vi "Transfer Images Data to UI.vi"(0 "fpga interface in":refnum<k20>, 1 "'stop' notifier":refnum<notifier>, 2 "Auto Vision Config":T1, 3 "measure call context in":refnum<class "Measure Call Context.lvclass">, 5 "Active Channel":string[](array[string]), 11 "error in":errorcluster, 12 "References":T6, 13 "raw display notifier":refnum<notifier>) -> (4 "fpga interface out":refnum<k20>, 15 "error out":errorcluster)   [LabVIEW 2025, in "Automotive Vision.lvclass"]
doc: "Handles frame grabbing, and prepare data for sendig it to the UI."
uses:
  Automotive Vision.lvclass
  <vilib>/Plug-In SDKs/Measurements/Measure Call Context/Measure Call Context.lvclass
  <vilib>/rvi/interface/nirviReadWriteControl/nirviReadWriteControl.xnode
  ttashjia/GSE/Host/Common/GettingStarted_Common_148X_Host.lvlib
  ttashjia/GSE/Host/Common/Types/148x_Common_FPGA_Reference.ctl
  NiFpgaLv.dll
  <vilib>/Utility/error.llb/Error Cluster From Error Code.vi
  <vilib>/rvi/interface/Simulation/niFpgaSimulationCallBeginRW.vi
  <vilib>/rvi/errors/niLvFpgaAdjustHostInterfaceError.vi
  <instrlib>/FlexRIO/CSI-2/v2/Common/Types/LLP Data Type.ctl
  <instrlib>/FlexRIO/CSI-2/v2/Common/NI CSI-2 API Common v2.lvlib
  Automotive-Vision OOB Data Transfer/Automotive-Vision OOB Data Transfer.lvlib
  Measurement Results.ctl
  <resource>/objmgr/niflexrioapiChannel.rc
  <instrlib>/FlexRIO/API/Host/v1/NI FlexRIO API v1.lvlib
  <instrlib>/FlexRIO/API/Host/v1/NI FlexRIO/API/Get Property Reference - Fpga Small.vi
  <vilib>/vision/Image Controls.llb/IMAQ Image.ctl
  ttashjia/GSE/Host/Common/Types/RAW Interpretation for Display.ctl
  ttashjia/GSE/Host/Common/Types/Serial Channel Display Parameters.ctl
  embedded data item.ctl
  embedded data.ctl
  register.ctl
  autovision_config.ctl
panel:
  out "output cluster 2":T5={"ACQ. IN PROGRESS"=FALSE, "IMAGE PIXEL DATA"=[], "ACQ. DURATION (s)"=0.0, "SOURCE RATE (fps)"=0.0, "BYTES ACQUIRED"=0, "FRAME COUNT"=0, "POC VOLTAGE (V)"=0.0, "POC CURRENT (A)"=0.0, "ERROR"=FALSE, "STATE MESSAGE"="Initializing...", "IMAGE DATA"="", "OOB gRPC Port"=0, "HEIGHT"=0, "WIDTH"=0, "FRAME COUNT BYTES"=[], "REGISTERS"=[], "COUNT LENGTH"=0} {"BYTES ACQUIRED" format="%#.6p"}
  in  "output cluster":T5={"ACQ. IN PROGRESS"=FALSE, "IMAGE PIXEL DATA"=[], "ACQ. DURATION (s)"=0.0, "SOURCE RATE (fps)"=0.0, "BYTES ACQUIRED"=0, "FRAME COUNT"=0, "POC VOLTAGE (V)"=0.0, "POC CURRENT (A)"=0.0, "ERROR"=FALSE, "STATE MESSAGE"="Initializing...", "IMAGE DATA"="", "OOB gRPC Port"=0, "HEIGHT"=0, "WIDTH"=0, "FRAME COUNT BYTES"=[], "REGISTERS"=[], "COUNT LENGTH"=0} {"BYTES ACQUIRED" format="%#.6p"}
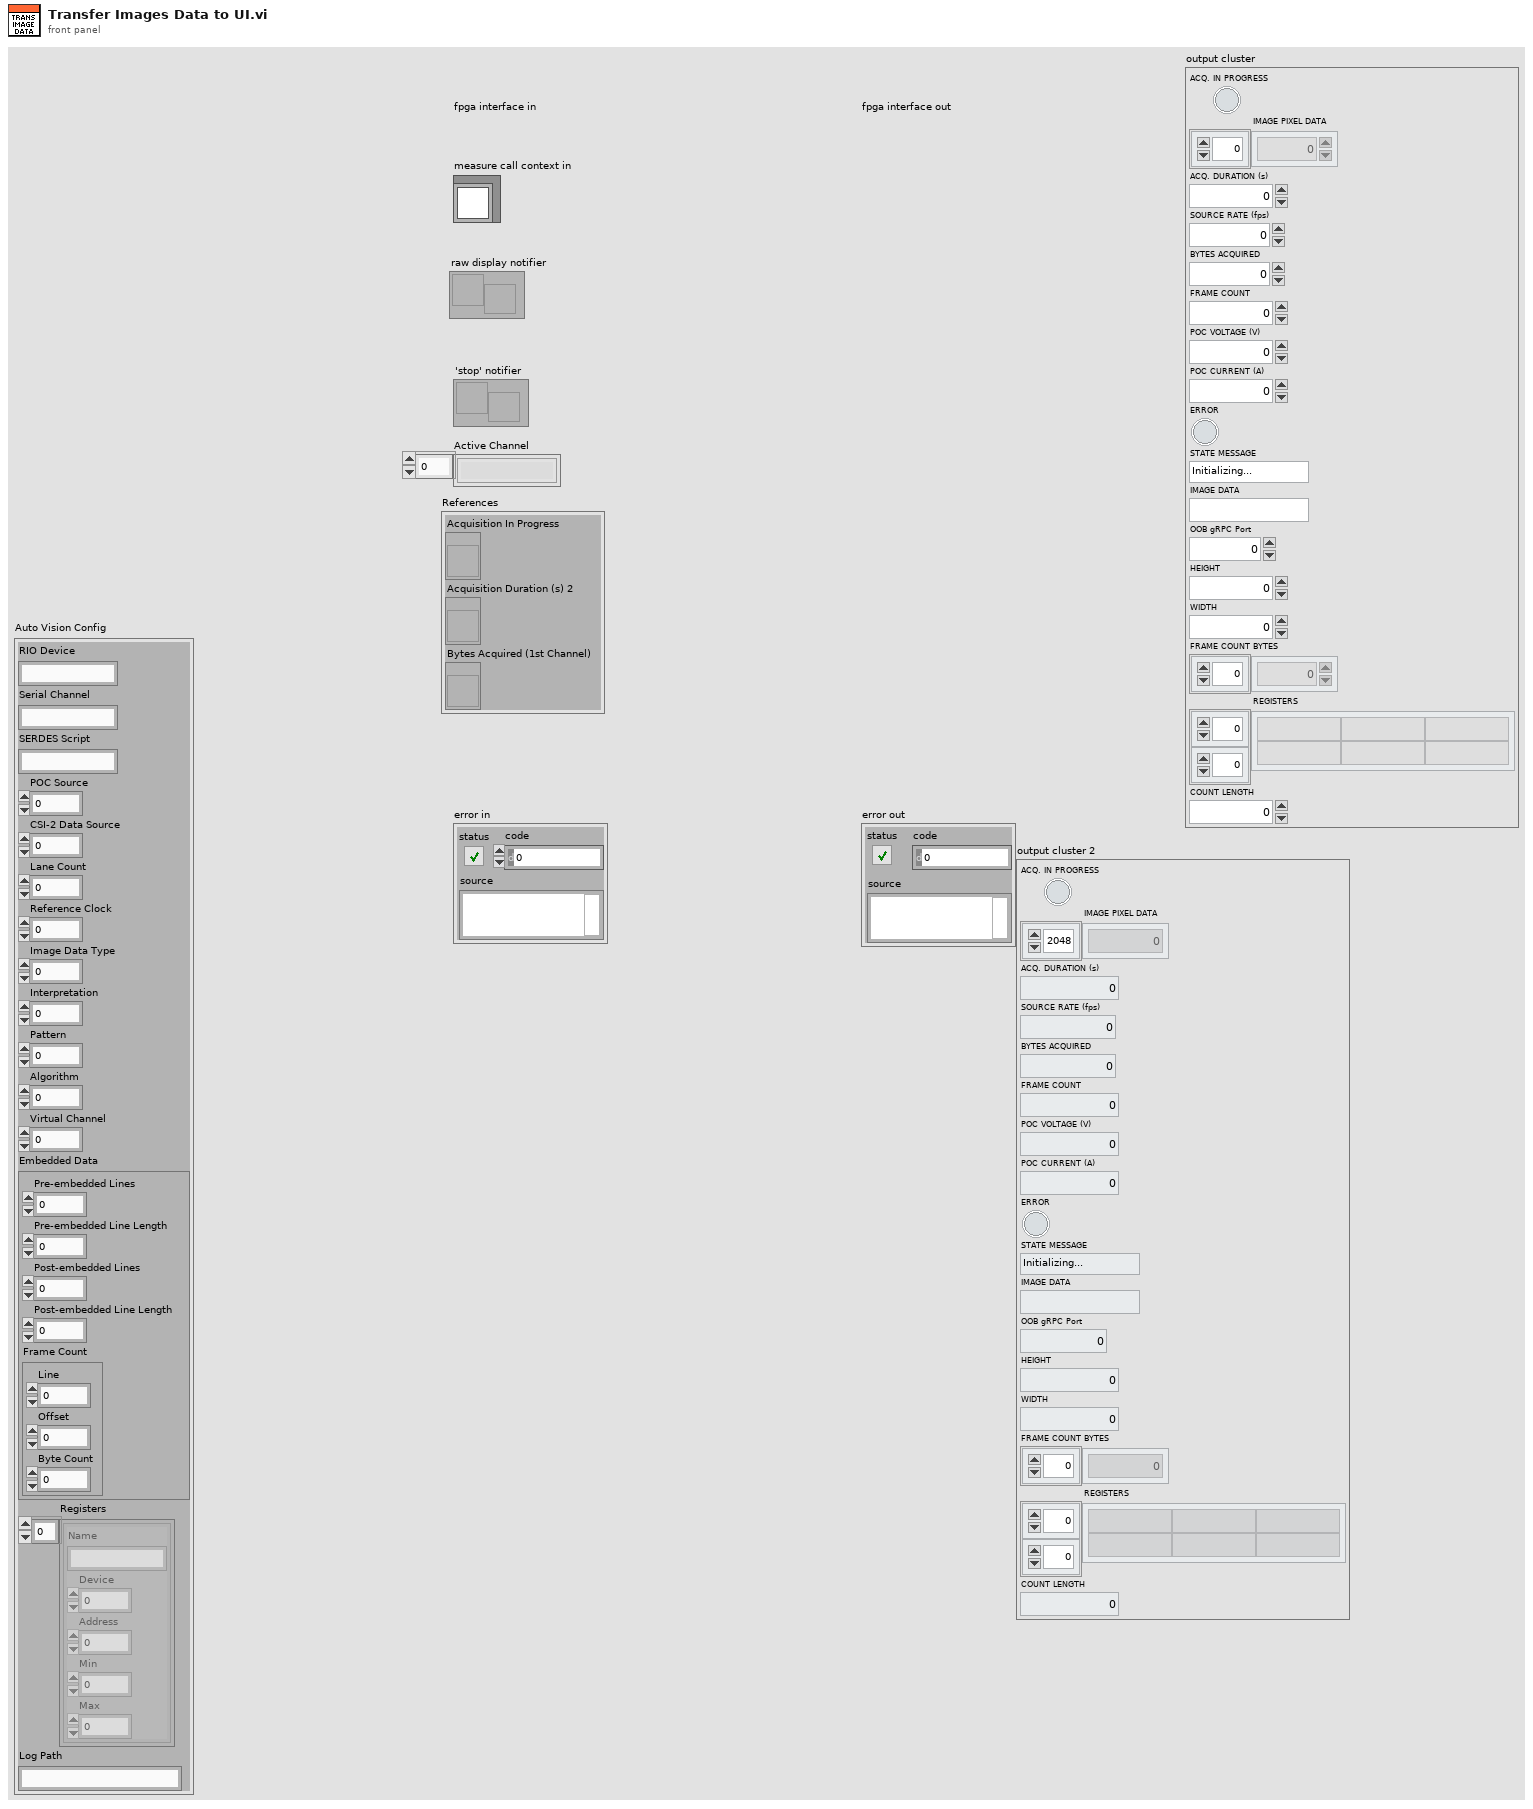
[diagram p1: front panel]
types:
  T1 = typedef "Automotive Vision.lvclass/autovision_config.ctl" = cluster{"RIO Device":string, "Serial Channel":string, "SERDES Script":string, "POC Source":u32, "CSI-2 Data Source":u32, "Lane Count":u32, "Reference Clock":dbl, "Image Data Type":u32, "Interpretation":u32, "Pattern":u32, "Algorithm":u32, "Virtual Channel":u32, "Embedded Data":T2, "Registers":T4[], "Log Path":string}
  T2 = typedef "Automotive Vision.lvclass/embedded data.ctl" = cluster{"Pre-embedded Lines":dbl, "Pre-embedded Line Length":dbl, "Post-embedded Lines":dbl, "Post-embedded Line Length":dbl, "Frame Count":T3}
  T3 = typedef "Automotive Vision.lvclass/embedded data item.ctl" = cluster{"Line":dbl, "Offset":dbl, "Byte Count":dbl}
  T4 = typedef "Automotive Vision.lvclass/register.ctl" = cluster{"Name":string, "Device":u8, "Address":u16, "Min":u16, "Max":u16}
  T5 = typedef "Automotive Vision.lvclass/Measurement Results.ctl" = cluster{"ACQ. IN PROGRESS":bool, "IMAGE PIXEL DATA":u32[], "ACQ. DURATION (s)":dbl, "SOURCE RATE (fps)":dbl, "BYTES ACQUIRED":u64, "FRAME COUNT":u64, "POC VOLTAGE (V)":dbl, "POC CURRENT (A)":dbl, "ERROR":bool, "STATE MESSAGE":string, "IMAGE DATA":string, "OOB gRPC Port":i32, "HEIGHT":u64, "WIDTH":u64, "FRAME COUNT BYTES":u32[], "REGISTERS":string[][], "COUNT LENGTH":u64}
  T6 = cluster{"Acquisition In Progress":refnum<vi>, "Acquisition Duration (s) 2":refnum<vi>, "Bytes Acquired (1st Channel)":refnum<vi>}
  T7 = typedef "NI CSI-2 API Common v2.lvlib/LLP Data Type.ctl" = enum8{"Frame Start", "Frame End", "Line Start", "Line End", "End of Transmission", "Reserved 0", "Reserved 1", "Reserved 2", "Generic Short Packet 1", "Generic Short Packet 2", "Generic Short Packet 3", "Generic Short Packet 4", "Generic Short Packet 5", "Generic Short Packet 6", "Generic Short Packet 7", "Generic Short Packet 8", "Null", "Blanking Data", "Embedded 8-bit non Image Data", "Generic Long Packet 1", "Generic Long Packet 2", "Generic Long Packet 3", "Generic Long Packet 4", "Reserved 3", "YUV420 8-bit", "YUV420 10-bit", "Legacy YUV420 8-bit", "Reserved 4", "YUV420 8-bit Chroma Shifted", "YUV420 10-bit Chroma Shifted", "YUV422 8-bit", "YUV422 10-bit", "RGB444", "RGB555", "RGB565", "RGB666", "RGB888", "Reserved 5", "Reserved 6", "RAW 24", "RAW 6", "RAW 7", "RAW 8", "RAW 10", "RAW 12", "RAW 14", "RAW 16", "RAW 20", "User Defined 8-bit Data 1", "User Defined 8-bit Data 2", "User Defined 8-bit Data 3", "User Defined 8-bit Data 4", "User Defined 8-bit Data 5", "User Defined 8-bit Data 6", "User Defined 8-bit Data 7", "User Defined 8-bit Data 8", "USL Command", "Reserved 7", "Reserved 8", "Reserved 9", "Reserved 10", "Reserved 11", "Reserved 12", "LRTE EPD Spacer"}
  T8 = cluster{"serial channel":fxp<+,3,3>, "frame number":u16, "data type":T7, "width":u16, "height":u16, "image bytes":u32, "total bytes":u32, "little endian":bool, "Status":string}
  T9 = typedef "GettingStarted_Common_148X_Host.lvlib/148x_Common_FPGA_Reference.ctl" = refnum<k20>
  T10 = typedef "GettingStarted_Common_148X_Host.lvlib/Serial Channel Display Parameters.ctl" = cluster{"images":cluster{"grayscale":T11, "color":T11}, "RAW parameters":cluster{"interpretation":T12, "bayer parameters":cluster{"pattern":i32, "algorithm":i32, "red gain":dbl, "green gain":dbl, "blue gain":dbl}}}
  T11 = typedef "IMAQ Image.ctl" = refnum<image>
  T12 = typedef "GettingStarted_Common_148X_Host.lvlib/RAW Interpretation for Display.ctl" = enum16{"Grayscale", "Bayer", "RGB", "YUV422", "YUV420", "Legacy YUV420"}
  T13 = typedef "GettingStarted_Common_148X_FPGA.lvlib/Image Metadata.ctl" = cluster{"serial channel":fxp<+,3,3>, "frame number":u16, "data type":T7, "width":u16, "height":u16, "image bytes":u32, "total bytes":u32, "little endian":bool}
  T14 = typedef "Automotive-Vision OOB Data Transfer.lvlib/OOB to Logic Data.ctl" = cluster{"PauseResume":bool, "ExportPath":string, "ExportType":u16, "Export":bool}
  T15 = cluster{"image pixel data fifo overflow":bool, "image metadata fifo overflow":bool}[]
  T16 = cluster{"image pixel data fifo overflow":bool, "image metadata fifo overflow":bool}
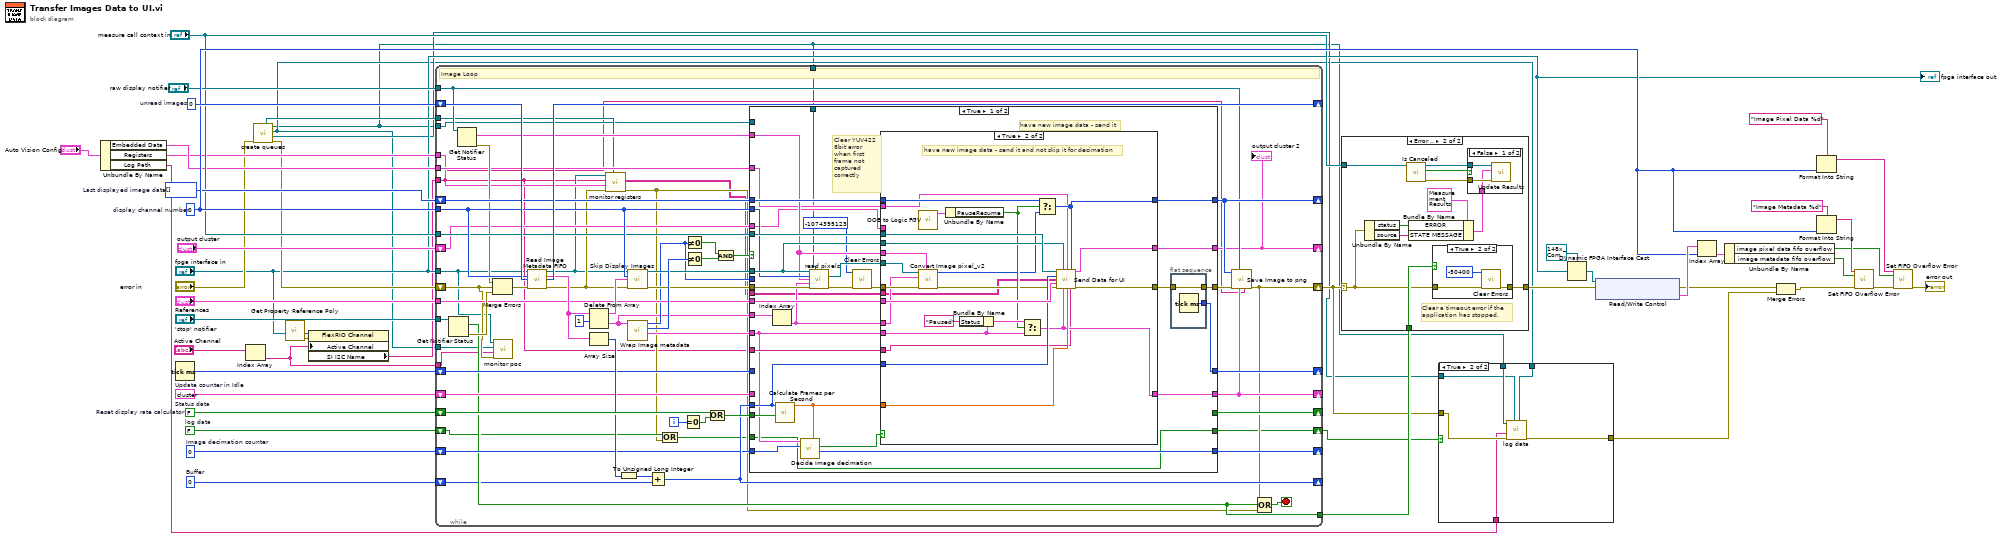
[diagram p0: block diagram]
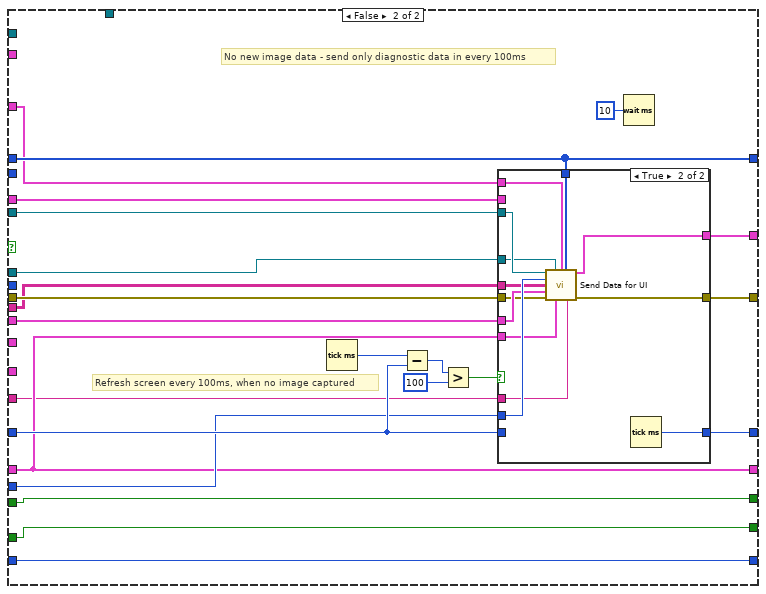
[diagram p4: hidden frame]
diagram:
  w16 = FALSE  # log data
  w26 = T8 {"serial channel"=0.0, "frame number"=0, "data type"=enum."Frame Start", "width"=0, "height"=0, "image bytes"=0, "total bytes"=0, "little endian"=FALSE, "Status"="Ready for Acquisition"}  # Status data
  w41 = 0  # display channel number
  w28 = u32 0  # Image decimation counter
  w29 = u32[] []  # Last displayed image data
  w33 = u32 0  # Buffer
  w34 = FALSE  # Reset display rate calculator
  w49 = u32 0  # unread images
  n1 = Unbundle By Name("Auto Vision Config") -> ("Embedded Data"=w21:T2, "Registers"=w20:T4[], "Log Path"=w5:string)
  n2 = Tick Count (ms) "Update counter in Idle"() -> (millisecond timer value=w30:u32)
  n3 = Index Array(array="Active Channel") -> (element=w3:string)  [unwired: 1 in]
  n4 = call "create queues.vi"("error in (no error)"="error in") -> ("error out"=w18:errorcluster, "i2c queue out"=w4:refnum<queue>, "power monitor queue out"=w2:refnum<queue>, "image queue out"=w1:refnum<queue>, "register monitor queue out"=w17:refnum<queue>)  [unwired: 6 in]
  n5 = call-poly <instrlib>:"Get Property Reference Poly.vi"("fpga interface in"="fpga interface in") -> ("error out"=w14:errorcluster, "property reference"=w13:refnum<k20>)  [unwired: 5 in, 1 out]
  n6 = property class="FlexRIO Channel"(reference=w13, error in=w14, "Active Channel"=w3) -> ("SI I2C Name"=w11:string)  [unwired: 2 out]
  n7 = while {
    shift-right: [w73] -> w7
    shift-left: w18 -> [w54]
    tunnel: "fpga interface in" -> [w52]
    shift-right: [w110] -> _
    shift-left: w49 -> [w101]
    tunnel: w41 -> [w90]
    shift-right: [w105] -> _
    shift-left: w34 -> [w102]
    shift-right: [w94] -> _
    shift-left: w33 -> [w77]
    tunnel: [w79] -> w32
    tunnel: "'stop' notifier" -> [w92]
    shift-right: [w88] -> _
    shift-left: w30 -> [w89]
    shift-right: [w76] -> _
    shift-left: w29 -> [w87]
    shift-right: [w85] -> _
    shift-left: w28 -> [w86]
    tunnel: "References" -> [w84]
    tunnel: "measure call context in" -> [w83]
    shift-right: [w74] -> _
    shift-left: w26 -> [w82]
    tunnel: "raw display notifier" -> [w72]
    tunnel: w21 -> [w68]
    shift-right: [w66] -> _
    shift-left: "output cluster" -> [w67]
    tunnel: w20 -> [w64]
    tunnel: w17 -> [w62]
    shift-right: [w56] -> w10
    shift-left: w16 -> [w61]
    tunnel: w1 -> [w58]
    tunnel: w11 -> [w55]
    tunnel: w3 -> [w53]
    tunnel: w2 -> [w51]
    tunnel: w1 -> [w50]
    i -> [w109]
    stop <- w111 stop-if-true
    # "Image Loop"
    n8 = Get Notifier Status(notifier=w92) -> (current notification=w79:bool, error out=w112:errorcluster)  [unwired: 1 in, 3 out]
    n9 = Get Notifier Status(notifier=w72) -> (current notification=w70:T10[], error out=w71:errorcluster)  [unwired: 1 in, 3 out]
    n10 = Merge Errors(w71, w54, w112) -> (w91:errorcluster)
    n11 = call "monitor poc.vi"("error in"=w54, "Active Channel"=w53, "power monitor queue in"=w51, "fpga interface in"=w52) -> ()  [unwired: 7 in, 1 out]
    n12 = call "Read Image Metadata FIFO.vi"("fpga inteface in"=w52, "display channel number"=w90, "number of images"=w101, "error in (no error)"=w91) -> ("fpga interface out"=w63:refnum<k20>, "image metadata"=w93:T13[], "images remaining"=w110:u32, "error out"=w65:errorcluster)  [unwired: 8 in]
    n13 = Delete From Array(array=w93, length=1) -> (deleted portion=w69:T13[], array with subset deleted=w96:T13[])  [unwired: 1 in]
    n14 = Array Size(array=w93) -> (size(s)=w95:i32)
    n15 = call "monitor registers.vi"("register monitor queue"=w62, "error in"=w65, "Registers"=w64, "bus instance name"=w55, "fpga interface in"=w63) -> ("error out"=w60:errorcluster, "registers out"=w57:string[][])  [unwired: 3 in, 2 out]
    n16 = To Unsigned Long Integer(number=w95) -> (unsigned 32bit integer=w78:u32)
    n17 = call "Skip Display Images.vi"("fpga interface in"=w63, "display channel number"=w90, "image metadata"=w96, "error in (no error)"=w65) -> ("fpga interface out"=w98:refnum<k20>, "error out"=w97:errorcluster)  [unwired: 10 in]
    n18 = call "Wrap Image metadata.vi"("image metadata"=w69) -> ("element"=w81:T8, "Numeric"=w100:i32, "total bytes"=w80:u32)  [unwired: 8 in]
    n19 = Add(x=w78, y=w77) -> (x+y=w94:u32)
    n20 = Compound Arithmetic op=OR(w61, w60) -> (w59:bool)
    n21 = Equal To 0?(x=w109) -> (x = 0?=w103:bool)
    n22 = Not Equal To 0?(x=w80) -> (x != 0?=w107:bool)
    n23 = Not Equal To 0?(x=w100) -> (x != 0?=w108:bool)
    n24 = Compound Arithmetic op=OR(w102, w103) -> (w104:bool)
    n25 = Compound Arithmetic op=AND(w107, w108) -> (w106:bool)
    n26 = case shown="True" w106 {
      tunnel: w97 -> [w130 w182]
      tunnel: w98 -> [w129 w180]
      tunnel: w90 -> [w128 _]
      tunnel: [w142 w189] -> w75
      tunnel: w104 -> [w133 w196]
      tunnel: [_ w196] -> w105
      tunnel: w94 -> [w139 w186]
      tunnel: w80 -> [_ _]
      tunnel: w81 -> [w123 _]
      tunnel: w83 -> [w144 w183]
      tunnel: w84 -> [w143 w197]
      tunnel: w89 -> [_ w188]
      tunnel: [w141 w190] -> w88
      tunnel: w87 -> [w138 w187]
      tunnel: [w140 w187] -> w76
      tunnel: w86 -> [w137 w185]
      tunnel: [w136 w185] -> w85
      tunnel: w82 -> [_ w184]
      tunnel: [w134 w184] -> w74
      tunnel: w55 -> [w132 w181]
      tunnel: w70 -> [w124 _]
      tunnel: w69 -> [w127 _]
      tunnel: w68 -> [w118 w179]
      tunnel: w67 -> [w116 w177]
      tunnel: [w117 w178] -> w66
      tunnel: w59 -> [w114 w175]
      tunnel: w58 -> [_ _]
      tunnel: w57 -> [w115 w176]
      tunnel: [w114 w175] -> w56
      tunnel: w50 -> [w113 _]
      frame True {
        # "Clear YUV422 8bit error when first frame not captured correctly"
        # "have new image data - send it"
        n27 = Index Array(array=w127) -> (element=w126:T13)  [unwired: 1 in]
        n28 = call <vilib>:"Calculate Frames per Second.vi"("Reset"=w133, "Buffer Number"=w139) -> ("Acquired Frames/s"=w122:dbl)  [unwired: 7 in, 2 out]
        n29 = call "Decide Image decimation.vi"("FPS"=w122, "Image decimation counter in"=w137, "element in"=w123) -> ("Image decimation counter out"=w136:u32, "send current image data"=w135:bool)  [unwired: 7 in]
        n30 = call "read pixels.vi"("fpga interface in"=w129, "image queue in"=w113, "display channel number"=w128, "serial channel display parameters"=w124, "image metadata"=w126, "error in (no error)"=w130) -> ("display image"=w125:T11, "error out"=w120:errorcluster)  [unwired: 7 in, 1 out]
        n31 = call <vilib>:"Clear Errors.vi"("error in (no error)"=w120, "specific error code to clear (0: all)"=-1074395123) -> ("error out"=w119:errorcluster)  [unwired: 4 in, 1 out]
        n32 = case shown="True" w135 {
          tunnel: [w146 w164] -> w131
          tunnel: w122 -> [_ w172]
          tunnel: w123 -> [w147 w159]
          tunnel: w144 -> [_ w171]
          tunnel: w143 -> [_ w170]
          tunnel: [w148 w169] -> w140
          tunnel: w139 -> [_ w168]
          tunnel: w138 -> [w148 w167]
          tunnel: [w147 w166] -> w134
          tunnel: w129 -> [_ w165]
          tunnel: w132 -> [_ w158]
          tunnel: w119 -> [w146 w157]
          tunnel: w125 -> [_ w155]
          tunnel: w126 -> [_ w153]
          tunnel: w124 -> [_ w152]
          tunnel: w118 -> [_ w151]
          tunnel: [w145 w150] -> w117
          tunnel: w116 -> [w145 _]
          tunnel: w115 -> [_ w149]
          frame False {
            # "have new image data - but skip the sending to not overload UI with data transfer"
          }
          frame True {
            # "have new image data - send it and not skip it for decimation"
            n33 = call "OOB to Logic FGV.vi"() -> ("OOB to Logic Data out"=w161:T14)  [unwired: 10 in, 1 out]
            n34 = call "Convert Image pixel_v2.vi"("serial channel display parameters"=w152, "error in"=w157, "image metadata"=w153, "Refnum in"=w155) -> ("error out"=w156:errorcluster, "Image Pixels (U32)"=w154:u32[])  [unwired: 6 in]
            n35 = Unbundle By Name(w161) -> ("PauseResume"=w160:bool)
            n36 = Bundle By Name(cluster=w159, "Status"="Paused") -> (w163:T8)
            n37 = Select(t=w163, s=w160, f=w159) -> (s? t:f=w166:T8)
            n38 = Select(t=w167, s=w160, f=w154) -> (s? t:f=w169:u32[])
            n39 = call "Send Data for UI.vi"("Measure Call Context in"=w171, "fpga interface in"=w165, "Embedded Data"=w151, "Last displayed image data"=w169, "FrameCount"=w168, "registers"=w149, "References"=w170, "error in"=w156, "Status data"=w166, "SOURCE RATE (fps)"=w172, "Active Channel"=w158) -> ("output cluster"=w150:T5, "error out"=w164:errorcluster)  [unwired: 3 in]
          }
        }
        n40 = flat-sequence {
          tunnel: [w174] -> w142
          tunnel: w131 -> [w174]
          tunnel: [w173] -> w141
          frame #0 {
            n41 = Tick Count (ms)() -> (millisecond timer value=w173:u32)
          }
        }
      }
      frame False {
        # "Refresh screen every 100ms, when no image captured"
        # "No new image data - send only diagnostic data in every 100ms"
        n42 = Tick Count (ms)() -> (millisecond timer value=w194:u32)
        n43 = Subtract(x=w194, y=w188) -> (x-y=w193:u32)
        n44 = Greater?(x=w193, y=u32 100) -> (0:w191:bool)
        n45 = case shown="True" w191 {
          tunnel: w182 -> [w200 w206]
          tunnel: [w200 w213] -> w189
          tunnel: w184 -> [_ w208]
          tunnel: w197 -> [_ w209]
          tunnel: [w199 w212] -> w190
          tunnel: w188 -> [w199 _]
          tunnel: w187 -> [_ w211]
          tunnel: w186 -> [_ w210]
          tunnel: w183 -> [_ w207]
          tunnel: w181 -> [_ w205]
          tunnel: w180 -> [_ w204]
          tunnel: w179 -> [_ w203]
          tunnel: [w198 w202] -> w178
          tunnel: w177 -> [w198 _]
          tunnel: w176 -> [_ w201]
          frame False {
          }
          frame True {
            n46 = call "Send Data for UI.vi"("Measure Call Context in"=w207, "fpga interface in"=w204, "Embedded Data"=w203, "Last displayed image data"=w211, "FrameCount"=w210, "registers"=w201, "References"=w209, "error in"=w206, "Status data"=w208, "Active Channel"=w205) -> ("output cluster"=w202:T5, "error out"=w213:errorcluster)  [unwired: 4 in]
            n47 = Tick Count (ms)() -> (millisecond timer value=w212:u32)
          }
        }
        n48 = Wait (ms)(milliseconds to wait=u32 10) -> ()  [unwired: 1 out]
      }
    }
    "output cluster 2" <- w66
    n49 = call "Save Image to png.vi"("Channel"=w55, "image metadata"=w74, "raw display notifier"=w72, "error in"=w75, "Last displayed image data"=w76) -> ("error out"=w73:errorcluster)  [unwired: 6 in]
    n50 = Compound Arithmetic op=OR(w73, w79, w60) -> (w111:bool)
  }
  n51 = case shown="Error .." w7 {
    selector: w7 -> [w214 w218]
    tunnel: [w214 w225] -> w44
    tunnel: w32 -> [_ w224]
    tunnel: "measure call context in" -> [_ w215]
    frame No Error {
    }
    frame Error {
      # "Clear a timeout error if the application has stopped."
      n52 = Unbundle By Name(w218) -> ("status"=w217:bool, "source"=w216:string)
      n53 = call <vilib>:"Is Canceled.vi"("measure call context in"=w215) -> ("error out"=w222:errorcluster, "is canceled?"=w221:bool, "measure call context out"=w223:refnum<class "Measure Call Context.lvclass">)  [unwired: 8 in]
      n54 = Bundle By Name(cluster=T5 {"ACQ. IN PROGRESS"=FALSE, "IMAGE PIXEL DATA"=[], "ACQ. DURATION (s)"=0.0, "SOURCE RATE (fps)"=0.0, "BYTES ACQUIRED"=0, "FRAME COUNT"=0, "POC VOLTAGE (V)"=0.0, "POC CURRENT (A)"=0.0, "ERROR"=FALSE, "STATE MESSAGE"="", "IMAGE DATA"="", "OOB gRPC Port"=0, "HEIGHT"=0, "WIDTH"=0, "FRAME COUNT BYTES"=[], "REGISTERS"=[], "COUNT LENGTH"=0} ("Measurement Results"), "ERROR"=w217, "STATE MESSAGE"=w216) -> (w219:T5)
      n55 = case shown="True" w224 {
        tunnel: w218 -> [w229 w232]
        tunnel: [w229 w230] -> w225
        frame False {
        }
        frame True {
          n56 = call <vilib>:"Clear Errors.vi"("error in (no error)"=w232, "specific error code to clear (0: all)"=-50400 ("y")) -> ("error out"=w230:errorcluster)  [unwired: 4 in, 1 out]
        }
      }
      n57 = case shown="False" w221 {
        tunnel: w223 -> [w228 _]
        tunnel: w222 -> [w227 _]
        tunnel: w219 -> [w226 _]
        frame False {
          n58 = call <vilib>:"Update Results.vi"("error in"=w227, "measurement results"=w226, "measure call context in"=w228) -> ()  [unwired: 7 in, 2 out]
        }
        frame True {
        }
      }
    }
  }
  n59 = case shown="True" w10 {
    tunnel: w7 -> [w233 w239]
    tunnel: [w233 w238] -> w6
    tunnel: w5 -> [_ w237]
    tunnel: w2 -> [_ w236]
    tunnel: w1 -> [_ w235]
    tunnel: w4 -> [_ w234]
    frame False {
    }
    frame True {
      n60 = call "log data.vi"("power monitor queue in"=w236, "i2c queue in"=w234, "error in"=w239, "path"=w237, "image queue in"=w235) -> ("error out"=w238:errorcluster)  [unwired: 6 in]
    }
  }
  n61 = Dynamic FPGA Interface Cast(Session In=T9 refnum ("FPGA VI Reference Out"), Type="fpga interface in") -> (Session Out=w45:T9)
  n62 = xnode ("Read/Write Control")("FPGA VI Reference In"=w45, "error in"=w44) -> ("error out"=w9:errorcluster, "display channel status"=w47:T15)  [unwired: 1 out]
  n63 = Index Array(array=w47, index=w41) -> (element=w48:T16)
  n64 = Unbundle By Name(w48) -> ("image pixel data fifo overflow"=w36:bool, "image metadata fifo overflow"=w35:bool)
  n65 = Merge Errors(w9, w6) -> (w8:errorcluster)
  n66 = Format Into String(format string="Image Pixel Data %d", w41) -> (resulting string=w38:string)  [unwired: 2 in, 1 out]
  n67 = Format Into String(format string="Image Metadata %d", w41) -> (resulting string=w37:string)  [unwired: 2 in, 1 out]
  n68 = call "Set FIFO Overflow Error.vi"("fifo name"=w37, "overflow"=w35, "error in (no error)"=w8) -> ("error out"=w40:errorcluster)  [unwired: 12 in]
  n69 = call "Set FIFO Overflow Error.vi"("fifo name"=w38, "overflow"=w36, "error in (no error)"=w40) -> ("error out"=→"error out":errorcluster)  [unwired: 12 in]
  "fpga interface out" <- "fpga interface in"
